vi "RThost.vi"() -> ()   [LabVIEW 2016]
uses:
  <vilib>/Utility/RT CPU Load.ctl
  Controls/StatesCIM.ctl
  Controls/srcmODE.ctl
  <vilib>/FPGAPlugInAG/cRIO-9068/niLvFpga_Open_cRIO-9068.vi
  <vilib>/rvi/interface/common/dynamic/niFpgaDynamicAddResources.vi
  <vilib>/Utility/error.llb/Error Cluster From Error Code.vi
  <vilib>/rvi/errors/niLvFpgaAdjustHostInterfaceError.vi
  <vilib>/FPGAPlugInAG/Dynamic/niLvFpga_Run_Dynamic.vi
  <vilib>/FPGAPlugInAG/Dynamic/niLvFpga_Reset_Dynamic.vi
  <vilib>/rvi/interface/nirviOpenFPGA/nirviOpenFPGA.xnode
  FPGA Bitfiles/CIMfpgaVI_BITFILE.lvbitx
  <vilib>/rvi/interface/nirviReadWriteControl/nirviReadWriteControl.xnode
  <vilib>/rvi/interface/nirviMethod/nirviMethod.xnode
  <vilib>/NI_Real-Time Target Support.lvlib
  NiFpgaLv.dll
  <vilib>/rvi/interface/Simulation/niFpgaSimulationCallBeginRW.vi
panel:
  out "ACCT current":fxp<+/-,24,5>
  out "Vmon current":fxp<+/-,24,5>
  out "DUTY Bad Cycles":u32
  out "VMONOff_READBACK":fxp<+/-,24,5>=-1.0
  out "ACCTThr_READBACK":fxp<+/-,24,5>=0.5
  out "VMONThr_READBACK":fxp<+/-,24,5>=-3.0
  out "SRCDuty":fxp<+,32,32>
  out "SRCPulse":u32
  out "acct prearm":fxp<+/-,24,5>
  out "vmon prearm":fxp<+/-,24,5>
  out "ACCT prearm MIN":fxp<+/-,24,5>
  out "vmon prearm MIN":fxp<+/-,24,5>
  out "vmon prearm MAX":fxp<+/-,24,5>
  out "ACCT prearm MAX":fxp<+/-,24,5>
  in  "Restart FPGA?":bool
  out "SRC:SVL:D2OpenStat":bool
  out "SRC:SVL:H2OpenStat":bool
  out "current state":T1(ring)
  out "State machine iterations":u32 caption="RUNNING"
  out "Running":bool
  out "Mode Error":errorcluster
  out "State Diag":T2
  out "Beam Mode":T3(ring)
  out "error IO":errorcluster
  out "init error":errorcluster
  out "chopper gate":bool
  out "Faraday":bool
  out "chopper OK":bool
  out "acct gateon":fxp<+/-,24,5>
  out "vmon gateon":fxp<+/-,24,5>
  out "acct gateoff":fxp<+/-,24,5>
  out "Vmon gateoff":fxp<+/-,24,5>
  out "FBIs":u32
  out "VMon Diag":fxp<+/-,24,5>
  out "ACCT Diag":fxp<+/-,24,5>
  out "Faraday Diag":bool
  out "C.GATE Diag":bool
  out "Duty Diag":bool
  out "Pulse Diag":bool
  in  "FPGA Read delay (ms)":u32=100
  in  "Refresh rate":dbl=1.0 caption="Delay Time (s)"
  out "CPU loads":T4[](array[typedef]) {"ISR (%)" format="%#.2f"; "Idle (%)" format="%#.2f"; "Background (%)" format="%#.2f"; "Normal (%)" format="%#.2f"; "Above Normal (%)" format="%#.2f"; "High (%)" format="%#.2g"; "Timed Structures (%)" format="%#.2g"; "Time Critical (%)" format="%#.2g"; "Total (%)" format="%#.2g"}
  out "# of CPUs":u32
  out "FBI":bool=TRUE
  # "cRIO LV RT Front Panel"
  # "EPICS CA"
  # "cRIO HW stats"
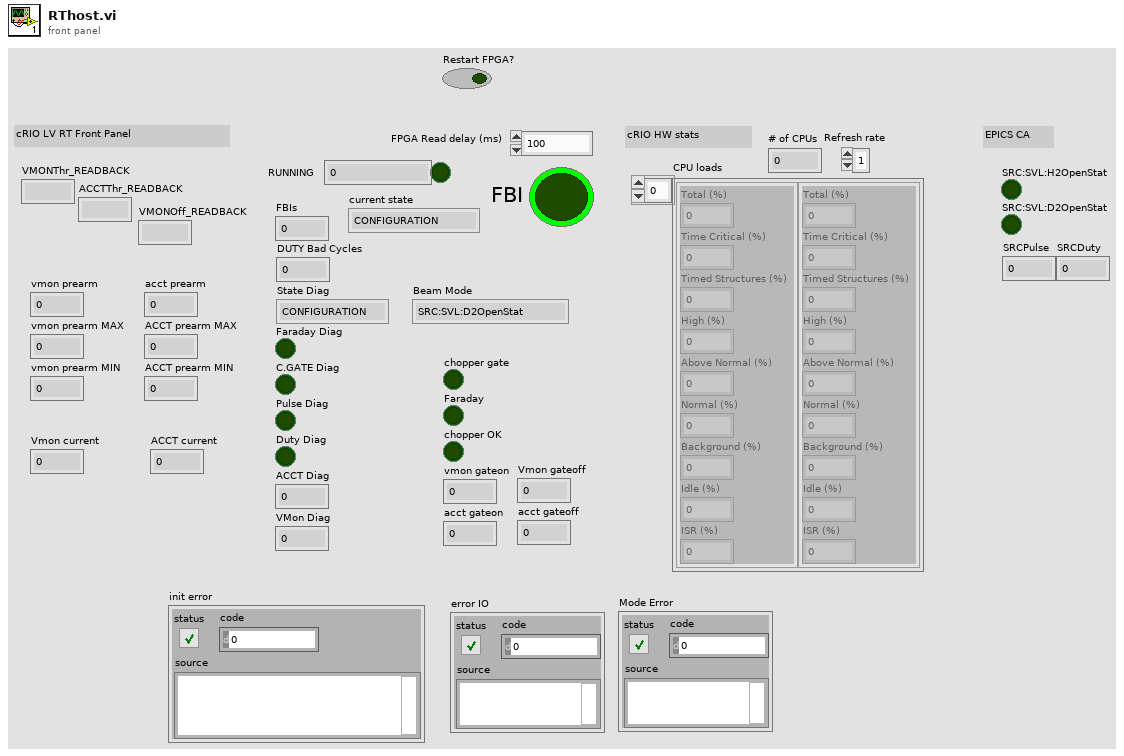
[diagram p1: front panel]
types:
  T1 = enum16{"CONFIGURATION", "PRE-ARM", "ARMED", "GATE OFF", "GATE ON: RISING", "GATE ON", "GATE OFF: DECREASING"}
  T2 = typedef "StatesCIM.ctl" = enum16{"CONFIGURATION", "PRE-ARM", "ARMED", "GATE OFF", "GATE ON: RISING", "GATE ON", "GATE OFF: DECREASING"}
  T3 = enum16{"SRC:SVL:D2OpenStat", "SRC:SVL:H2OpenStat"}
  T4 = typedef "NI_Real-Time Target Support.lvlib/RT CPU Load.ctl" = cluster{"Total (%)":dbl, "Time Critical (%)":dbl, "Timed Structures (%)":dbl, "High (%)":dbl, "Above Normal (%)":dbl, "Normal (%)":dbl, "Background (%)":dbl, "Idle (%)":dbl, "ISR (%)":dbl}
  T5 = typedef "srcmODE.ctl" = enum16{"SRC:SVL:D2OpenStat", "SRC:SVL:H2OpenStat"}
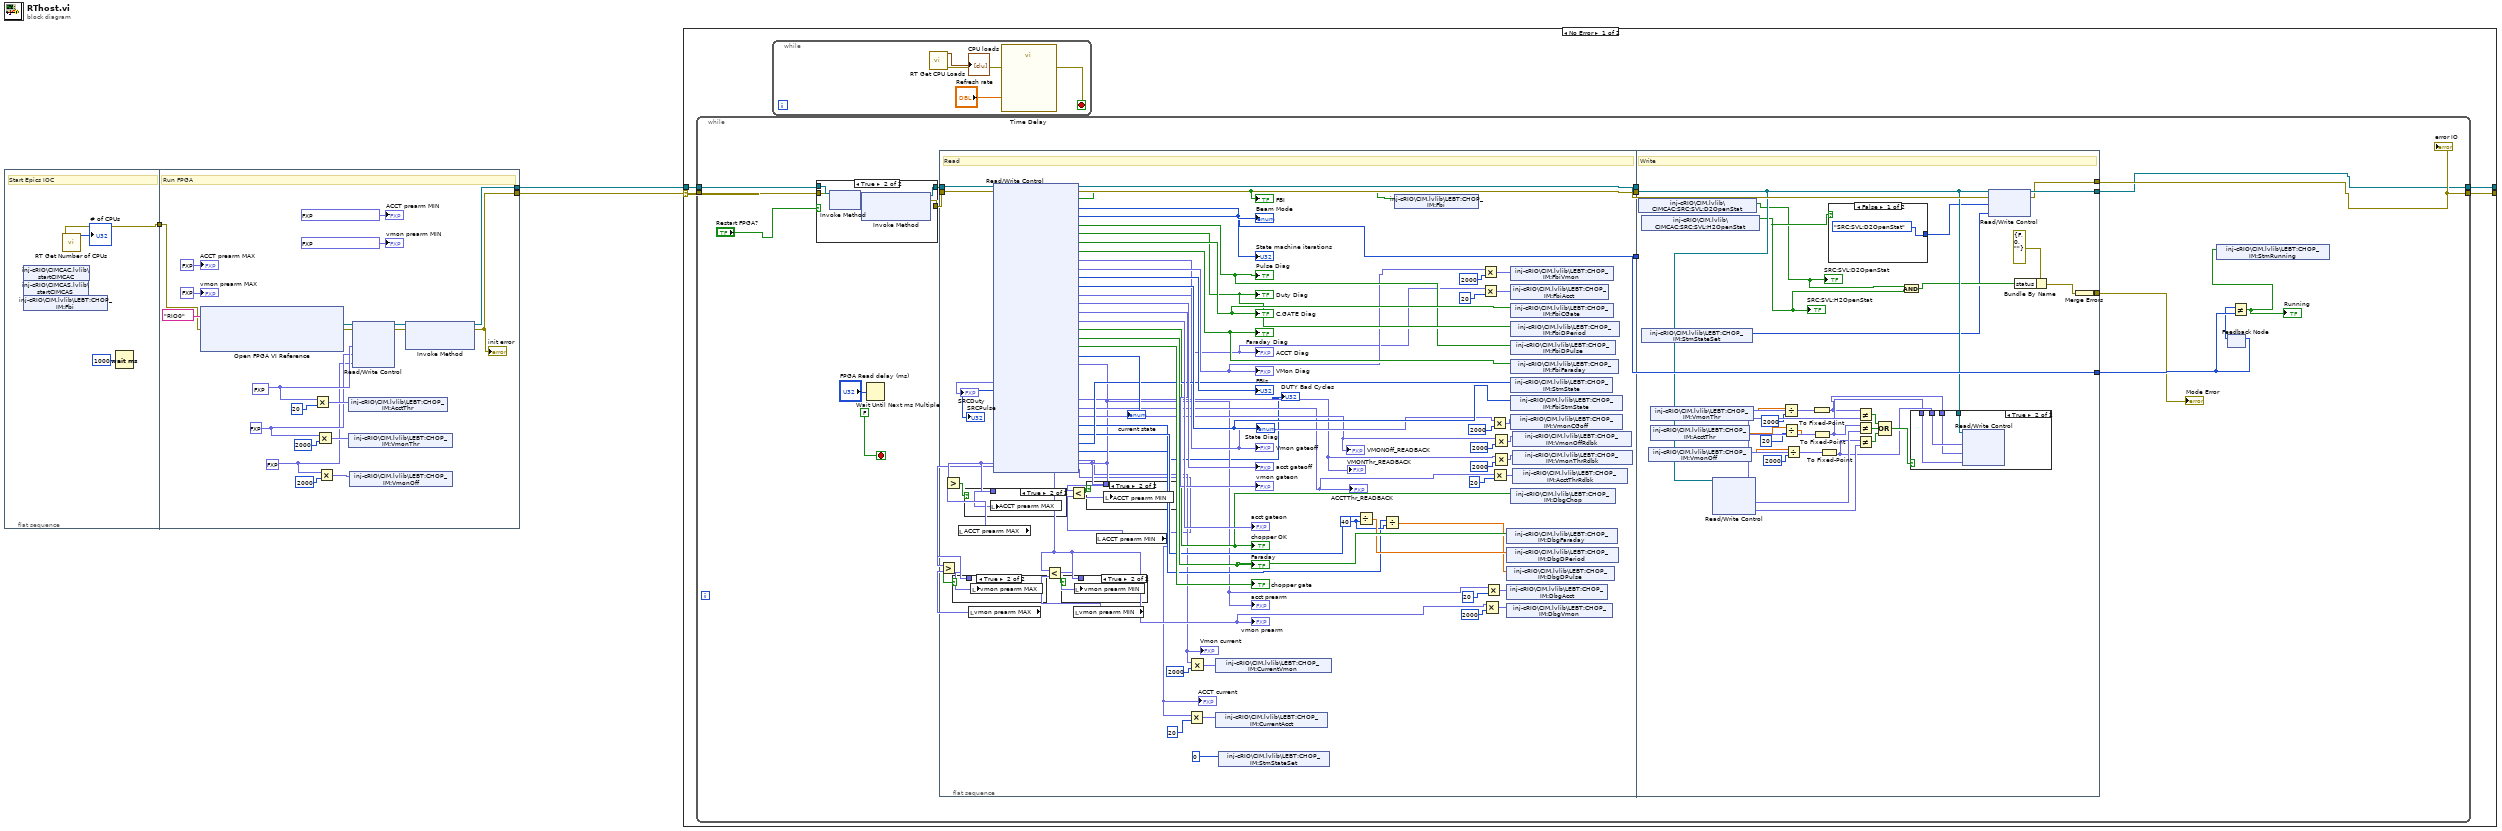
[diagram p0: block diagram]
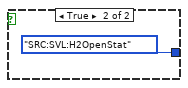
[diagram p7: hidden frame]
diagram:
  n1 = flat-sequence {
    tunnel: [w5] -> w3
    tunnel: w3 -> [w26]
    tunnel: [w20] -> w1
    tunnel: [w21] -> w2
    frame #0 {
      # "Start Epics IOC"
      n2 = shared-variable "inj-cRIO\\CIMCAC.lvlib\\startCIMCAC"() -> ()  [unwired: 1 in, 2 out]
      n3 = shared-variable "inj-cRIO\\CIMCAS.lvlib\\startCIMCAS"() -> ()  [unwired: 1 in, 2 out]
      n4 = shared-variable "inj-cRIO\\CIM.lvlib\\LEBT:CHOP_IM:Fbi"() -> ()  [unwired: 1 in, 2 out]
      n5 = call <vilib>:"RT Get Number of CPUs.vi"() -> ("error out"=w5:errorcluster, "# of CPUs"=→"# of CPUs":u32)  [unwired: 10 in]
      n6 = Wait (ms)(milliseconds to wait=u32 1000) -> ()  [unwired: 1 out]
    }
    frame #1 {
      w7 = fxp<+/-,24,5> 0.5 ("ACCTThr")
      w9 = fxp<+/-,24,5> 3.0 ("VMONThr")
      w12 = fxp<+/-,24,5> 0.25 ("VMONOff")
      # "Run FPGA"
      n7 = xnode "Open FPGA VI Reference"("error in"=w26, "resource name"=tag "RIO0") -> ("FPGA VI Reference Out"=w16:refnum<k20>, "error out"=w17:errorcluster)
      n8 = Multiply(x=w12, y=20) -> (x*y=w10:fxp<+/-,56,37>)
      n9 = Multiply(x=w9, y=2000) -> (x*y=w8:fxp<+/-,56,37>)
      n10 = Multiply(x=w7, y=2000) -> (x*y=w13:fxp<+/-,56,37>)
      n11 = shared-variable "inj-cRIO\\CIM.lvlib\\LEBT:CHOP_IM:AcctThr"(w10) -> ()  [unwired: 1 in, 1 out]
      n12 = shared-variable "inj-cRIO\\CIM.lvlib\\LEBT:CHOP_IM:VmonThr"(w8) -> ()  [unwired: 1 in, 1 out]
      n13 = shared-variable "inj-cRIO\\CIM.lvlib\\LEBT:CHOP_IM:VmonOff"(w13) -> ()  [unwired: 1 in, 1 out]
      n14 = xnode "Read/Write Control"("FPGA VI Reference In"=w16, "error in"=w17, "ACCTThr"=w12, "VMONThr"=w9, "VMONOff"=w7) -> ("FPGA VI Reference Out"=w19:refnum<k20>, "error out"=w18:errorcluster)  [unwired: 1 out]
      n15 = xnode "Invoke Method"("FPGA VI Reference In"=w19, "error in"=w18) -> ("FPGA VI Reference Out"=w21:refnum<k20>, "error out"=w20:errorcluster)  [unwired: 1 in]
      "init error" <- w20
      "ACCT prearm MAX" <- fxp<+/-,24,5> -16.0 ("ACCT prearm MAX")
      "ACCT prearm MIN" <- fxp<+/-,24,5> 15.999998092651367 ("ACCT prearm MIN")
      "vmon prearm MIN" <- fxp<+/-,24,5> 15.999998092651367 ("vmon prearm MIN")
      "vmon prearm MAX" <- fxp<+/-,24,5> -16.0 ("vmon prearm MAX")
    }
  }
  n16 = case shown="No Error" w1 {
    selector: w1 -> [w28 w170]
    tunnel: [w31 w169] -> _
    tunnel: [w30 w170] -> _
    tunnel: w2 -> [w29 w169]
    frame No Error {
      n17 = while {
        tunnel: w29 -> [w42]
        tunnel: w28 -> [w43]
        tunnel: [w36] -> w31
        tunnel: [w37] -> w30
        stop <- FALSE stop-if-true
        n18 = case shown="True" "Restart FPGA?" {
          tunnel: w43 -> [w51 w53]
          tunnel: w42 -> [w52 w58]
          tunnel: [w52 w54] -> w41
          tunnel: [w51 w55] -> w40
          frame False {
          }
          frame True {
            n19 = xnode "Invoke Method"("FPGA VI Reference In"=w58, "error in"=w53) -> ("FPGA VI Reference Out"=w56:refnum<k20>, "error out"=w57:errorcluster)
            n20 = xnode "Invoke Method"("FPGA VI Reference In"=w56, "error in"=w57) -> ("FPGA VI Reference Out"=w54:refnum<k20>, "error out"=w55:errorcluster)  [unwired: 1 in]
          }
        }
        n21 = Wait Until Next ms Multiple(millisecond multiple="FPGA Read delay (ms)") -> ()  [unwired: 1 out]
        n22 = flat-sequence {
          tunnel: w40 -> [w126]
          tunnel: w41 -> [w125]
          tunnel: [w124] -> w48
          tunnel: [w123] -> w47
          tunnel: [w120] -> w46
          tunnel: w48 -> [w154]
          tunnel: w47 -> [w162]
          tunnel: w46 -> [w161]
          tunnel: [w161] -> w45
          tunnel: [w149] -> w38
          tunnel: [w147] -> w36
          tunnel: [w146] -> w37
          frame #0 {
            w93 = u32 40 ("y")
            # "Read"
            n23 = local read "ACCT prearm MAX"() -> (w109:fxp<+/-,24,5>)
            n24 = local read "vmon prearm MAX"() -> (w107:fxp<+/-,24,5>)
            n25 = xnode "Read/Write Control"("FPGA VI Reference In"=w125, "error in"=w126) -> ("FPGA VI Reference Out"=w124:refnum<k20>, "error out"=w123:errorcluster, "FBI"=w104:bool, "SRCMode"=→"Beam Mode":T3, "State machine iterations"=w120:u32, "Pulse Diag"=w101:bool, "Duty Diag"=w102:bool, "C.GATE Diag"=w103:bool, "Faraday Diag"=w100:bool, "ACCT Diag"=w76:fxp<+/-,24,5>, "VMon Diag"=w90:fxp<+/-,24,5>, "FBIs"=→"FBIs":u32, "State Diag"=w98:T1, "Vmon gateoff"=w85:fxp<+/-,24,5>, "acct gateoff"=→"acct gateoff":fxp<+/-,24,5>, "vmon gateon"=→"vmon gateon":fxp<+/-,24,5>, "acct gateon"=→"acct gateon":fxp<+/-,24,5>, "chopper OK"=w96:bool, "Faraday"=w99:bool, "chopper gate"=→"chopper gate":bool, "current state"=→"current state":T1, "acct prearm"=w70:fxp<+/-,24,5>, "vmon prearm"=w67:fxp<+/-,24,5>, "SRCDuty"=→"SRCDuty":fxp<+,32,32>, "SRCPulse"=→"SRCPulse":u32, "VMONThr_readback"=w79:fxp<+/-,24,5>, "ACCTThr_readback"=w73:fxp<+/-,24,5>, "VMONOff_readback"=w82:fxp<+/-,24,5>, "High Period (Ticks)"=w92:u32, "Low Period (Ticks)"=w95:u32, "current state"=w97:T1, "DUTY Bad Cycles"=→"DUTY Bad Cycles":u32, "Vmon current"=w61:fxp<+/-,24,5>, "ACCT current"=w60:fxp<+/-,24,5>)
            "FBI" <- w104
            "State machine iterations" <- w120
            "Pulse Diag" <- w101
            "Duty Diag" <- w102
            "C.GATE Diag" <- w103
            "Faraday Diag" <- w100
            "ACCT Diag" <- w76
            "VMon Diag" <- w90
            "Vmon gateoff" <- w85
            "chopper OK" <- w96
            "Faraday" <- w99
            "State Diag" <- w98
            "vmon prearm" <- w67
            "acct prearm" <- w70
            "VMONThr_READBACK" <- w79
            "ACCTThr_READBACK" <- w73
            "VMONOff_READBACK" <- w82
            "Vmon current" <- w61
            "ACCT current" <- w60
            n26 = Greater?(x=w67, y=w107) -> (0:w113:bool)
            n27 = Greater?(x=w70, y=w109) -> (0:w116:bool)
            n28 = case shown="True" w113 {
              tunnel: w67 -> [_ w129]
              frame False {
              }
              frame True {
                n29 = local write "vmon prearm MAX"(w129) -> ()
              }
            }
            n30 = case shown="True" w116 {
              tunnel: w70 -> [_ w130]
              frame False {
              }
              frame True {
                n31 = local write "ACCT prearm MAX"(w130) -> ()
              }
            }
            n32 = local read "vmon prearm MIN"() -> (w108:fxp<+/-,24,5>)
            n33 = Less?(x=w67, y=w108) -> (x < y?=w112:bool)
            n34 = case shown="True" w112 {
              tunnel: w67 -> [_ w128]
              frame False {
              }
              frame True {
                n35 = local write "vmon prearm MIN"(w128) -> ()
              }
            }
            n36 = local read "ACCT prearm MIN"() -> (w110:fxp<+/-,24,5>)
            n37 = Less?(x=w70, y=w110) -> (x < y?=w111:bool)
            n38 = case shown="True" w111 {
              tunnel: w70 -> [_ w127]
              frame False {
              }
              frame True {
                n39 = local write "ACCT prearm MIN"(w127) -> ()
              }
            }
            n40 = Multiply(x=w60, y=20) -> (x*y=w62:fxp<+/-,56,37>)
            n41 = Multiply(x=w61, y=2000) -> (x*y=w65:fxp<+/-,56,37>)
            n42 = shared-variable "inj-cRIO\\CIM.lvlib\\LEBT:CHOP_IM:CurrentVmon"(w65) -> ()  [unwired: 1 in, 1 out]
            n43 = shared-variable "inj-cRIO\\CIM.lvlib\\LEBT:CHOP_IM:CurrentAcct"(w62) -> ()  [unwired: 1 in, 1 out]
            n44 = shared-variable "inj-cRIO\\CIM.lvlib\\LEBT:CHOP_IM:StmStateSet"(0) -> ()  [unwired: 1 in, 1 out]
            n45 = Divide(x=w95, y=w93) -> (x/y=w94:dbl)
            n46 = Divide(x=w92, y=w93) -> (x/y=w91:dbl)
            n47 = shared-variable "inj-cRIO\\CIM.lvlib\\LEBT:CHOP_IM:Fbi"(w104) -> ()  [unwired: 1 in, 1 out]
            n48 = Multiply(x=w90, y=2000) -> (x*y=w88:fxp<+/-,56,37>)
            n49 = Multiply(x=w76, y=20) -> (x*y=w74:fxp<+/-,56,37>)
            n50 = Multiply(x=w67, y=2000) -> (x*y=w77:fxp<+/-,56,37>)
            n51 = Multiply(x=w70, y=20) -> (x*y=w68:fxp<+/-,56,37>)
            n52 = Multiply(x=w85, y=2000) -> (x*y=w87:fxp<+/-,56,37>)
            n53 = Multiply(x=w73, y=20) -> (x*y=w71:fxp<+/-,56,37>)
            n54 = Multiply(x=w82, y=2000) -> (x*y=w84:fxp<+/-,56,37>)
            n55 = Multiply(x=w79, y=2000) -> (x*y=w81:fxp<+/-,56,37>)
            n56 = shared-variable "inj-cRIO\\CIM.lvlib\\LEBT:CHOP_IM:DbgFaraday"(w99) -> ()  [unwired: 1 in, 1 out]
            n57 = shared-variable "inj-cRIO\\CIM.lvlib\\LEBT:CHOP_IM:DbgDPeriod"(w94) -> ()  [unwired: 1 in, 1 out]
            n58 = shared-variable "inj-cRIO\\CIM.lvlib\\LEBT:CHOP_IM:DbgDPulse"(w91) -> ()  [unwired: 1 in, 1 out]
            n59 = shared-variable "inj-cRIO\\CIM.lvlib\\LEBT:CHOP_IM:DbgAcct"(w68) -> ()  [unwired: 1 in, 1 out]
            n60 = shared-variable "inj-cRIO\\CIM.lvlib\\LEBT:CHOP_IM:DbgVmon"(w77) -> ()  [unwired: 1 in, 1 out]
            n61 = shared-variable "inj-cRIO\\CIM.lvlib\\LEBT:CHOP_IM:FbiVmon"(w88) -> ()  [unwired: 1 in, 1 out]
            n62 = shared-variable "inj-cRIO\\CIM.lvlib\\LEBT:CHOP_IM:FbiAcct"(w74) -> ()  [unwired: 1 in, 1 out]
            n63 = shared-variable "inj-cRIO\\CIM.lvlib\\LEBT:CHOP_IM:FbiCGate"(w103) -> ()  [unwired: 1 in, 1 out]
            n64 = shared-variable "inj-cRIO\\CIM.lvlib\\LEBT:CHOP_IM:FbiDPeriod"(w102) -> ()  [unwired: 1 in, 1 out]
            n65 = shared-variable "inj-cRIO\\CIM.lvlib\\LEBT:CHOP_IM:FbiDPulse"(w101) -> ()  [unwired: 1 in, 1 out]
            n66 = shared-variable "inj-cRIO\\CIM.lvlib\\LEBT:CHOP_IM:FbiFaraday"(w100) -> ()  [unwired: 1 in, 1 out]
            n67 = shared-variable "inj-cRIO\\CIM.lvlib\\LEBT:CHOP_IM:StmState"(w97) -> ()  [unwired: 1 in, 1 out]
            n68 = shared-variable "inj-cRIO\\CIM.lvlib\\LEBT:CHOP_IM:FbiStmState"(w98) -> ()  [unwired: 1 in, 1 out]
            n69 = shared-variable "inj-cRIO\\CIM.lvlib\\LEBT:CHOP_IM:VmonCGoff"(w87) -> ()  [unwired: 1 in, 1 out]
            n70 = shared-variable "inj-cRIO\\CIM.lvlib\\LEBT:CHOP_IM:DbgChop"(w96) -> ()  [unwired: 1 in, 1 out]
            n71 = shared-variable "inj-cRIO\\CIM.lvlib\\LEBT:CHOP_IM:VmonOffRdbk"(w84) -> ()  [unwired: 1 in, 1 out]
            n72 = shared-variable "inj-cRIO\\CIM.lvlib\\LEBT:CHOP_IM:VmonThrRdbk"(w81) -> ()  [unwired: 1 in, 1 out]
            n73 = shared-variable "inj-cRIO\\CIM.lvlib\\LEBT:CHOP_IM:AcctThrRdbk"(w71) -> ()  [unwired: 1 in, 1 out]
          }
          frame #1 {
            # "Write"
            n74 = shared-variable "inj-cRIO\\CIM.lvlib\\CIMCAC:SRC:SVL:D2OpenStat"() -> (w145:bool)  [unwired: 1 in, 1 out]
            "SRC:SVL:D2OpenStat" <- w145
            n75 = shared-variable "inj-cRIO\\CIM.lvlib\\CIMCAC:SRC:SVL:H2OpenStat"() -> (w152:bool)  [unwired: 1 in, 1 out]
            "SRC:SVL:H2OpenStat" <- w152
            n76 = shared-variable "inj-cRIO\\CIM.lvlib\\LEBT:CHOP_IM:StmStateSet"() -> (w131:u16)  [unwired: 1 in, 1 out]
            n77 = shared-variable "inj-cRIO\\CIM.lvlib\\LEBT:CHOP_IM:VmonOff"() -> (w137:dbl)  [unwired: 1 in, 1 out]
            n78 = shared-variable "inj-cRIO\\CIM.lvlib\\LEBT:CHOP_IM:VmonThr"() -> (w140:dbl)  [unwired: 1 in, 1 out]
            n79 = shared-variable "inj-cRIO\\CIM.lvlib\\LEBT:CHOP_IM:AcctThr"() -> (w134:dbl)  [unwired: 1 in, 1 out]
            n80 = xnode "Read/Write Control"("FPGA VI Reference In"=w154) -> ("VMONThr"=w143:fxp<+/-,24,5>, "ACCTThr"=w156:fxp<+/-,24,5>, "VMONOff"=w155:fxp<+/-,24,5>)  [unwired: 1 in, 2 out]
            n81 = Divide(x=w140, y=2000) -> (x/y=w138:dbl)
            n82 = Divide(x=w134, y=20) -> (x/y=w132:dbl)
            n83 = Divide(x=w137, y=2000) -> (x/y=w135:dbl)
            n84 = To Fixed-Point(fixed-point type=w143, number=w138) -> (fixed-point=w141:fxp<+/-,24,5>)
            n85 = To Fixed-Point(fixed-point type=w143, number=w132) -> (fixed-point=w142:fxp<+/-,24,5>)
            n86 = To Fixed-Point(fixed-point type=w143, number=w135) -> (fixed-point=w144:fxp<+/-,24,5>)
            n87 = case shown="False" w152 {
              tunnel: [srcmODE."SRC:SVL:D2OpenStat" ("SRCMode") srcmODE."SRC:SVL:H2OpenStat" ("SRCMode")] -> w153
              frame False {
              }
              frame True {
              }
            }
            n88 = Not Equal?(x=w141, y=w143) -> (x != y?=w159:bool)
            n89 = Not Equal?(x=w142, y=w156) -> (x != y?=w158:bool)
            n90 = Not Equal?(x=w144, y=w155) -> (x != y?=w157:bool)
            n91 = Compound Arithmetic op=OR(w159, w158, w157) -> (w160:bool)
            n92 = And(x=w145, y=w152) -> (x .and. y?=w151:bool)
            n93 = case shown="True" w160 {
              tunnel: w144 -> [_ w168]
              tunnel: w141 -> [_ w167]
              tunnel: w142 -> [_ w166]
              tunnel: w154 -> [_ w165]
              frame False {
              }
              frame True {
                n94 = xnode "Read/Write Control"("FPGA VI Reference In"=w165, "VMONOff"=w168, "VMONThr"=w167, "ACCTThr"=w166) -> ()  [unwired: 1 in, 2 out]
              }
            }
            n95 = xnode "Read/Write Control"("FPGA VI Reference In"=w154, "error in"=w162, "SRCMode"=w153, "State Set"=w131) -> ("FPGA VI Reference Out"=w147:refnum<k20>, "error out"=w146:errorcluster)
            n96 = Bundle By Name(cluster=errorcluster {"status"=FALSE, "code"=0, "source"=""} ("error out"), "status"=w151) -> (w150:errorcluster)
            n97 = Merge Errors(w150) -> (w149:errorcluster)
          }
        }
        n98 = feedback #1() -> (w44:u32)  [unwired: 1 in]
        n99 = feedback-in #1(w45) -> ()
        n100 = Not Equal?(x=w44, y=w45) -> (x != y?=w39:bool)
        "Running" <- w39
        n101 = shared-variable "inj-cRIO\\CIM.lvlib\\LEBT:CHOP_IM:StmRunning"(w39) -> ()  [unwired: 1 in, 1 out]
        "Mode Error" <- w38
        "error IO" <- w37
      }
      n102 = while {
        stop <- w33 stop-if-true
        n103 = call <vilib>:"RT Get CPU Loads.vi"() -> ("error out"=w33:errorcluster, "CPU loads"=→"CPU loads":T4[])  [unwired: 10 in]
        n104 = call "Time Delay"("Delay Time (s)"="Refresh rate") -> ()  [unwired: 10 in, 1 out]
      }
    }
    frame Error {
    }
  }
